vi "Requirement Coverage.vi"() -> ()   [LabVIEW 2013]
uses:
  <vilib>/addons/_JKI Toolkits/Caraya/classes/Test/Test.lvclass
  <vilib>/LabVIEW Open Source Project/MQTT TCP Connection/MQTT_TCP/Connection/TCPConnection.lvclass
  source/Server class/Server.lvclass
  <vilib>/LabVIEW Open Source Project/MQTT Connection/MQTT_Base/Base Class/MQTT_Base.lvclass
panel:
  out "error out":errorcluster
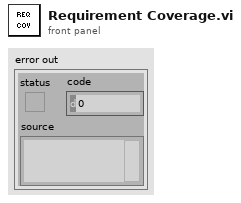
[diagram p1: front panel]
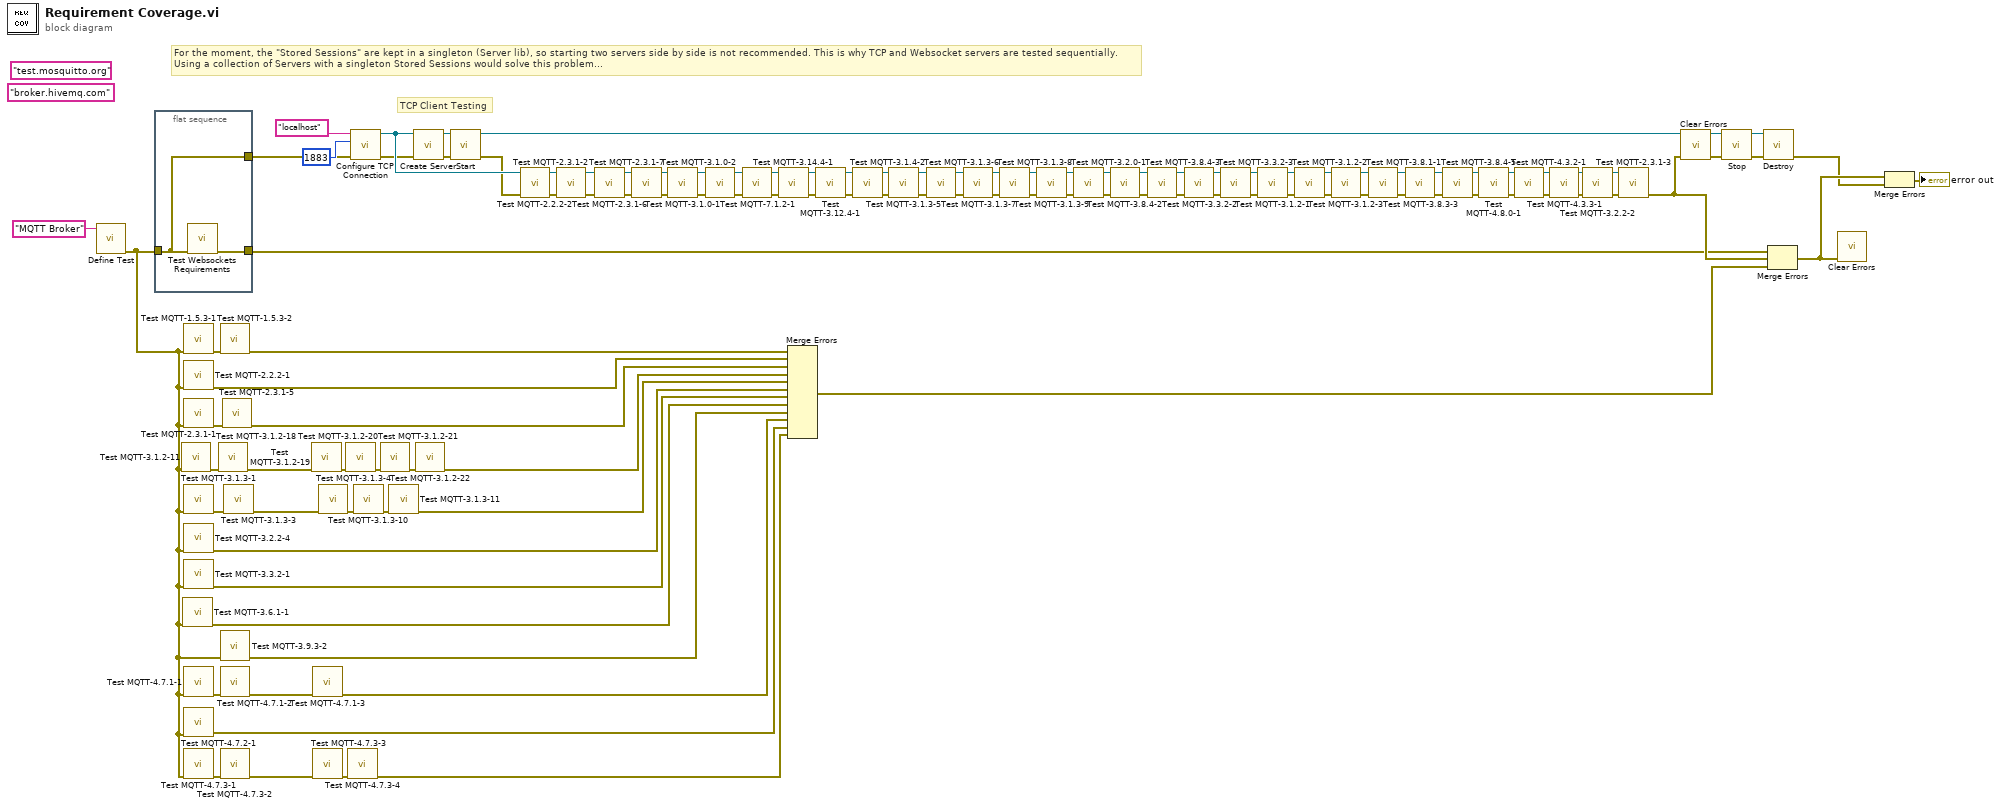
[diagram p0: block diagram]
diagram:
  (unwired) "test.mosquitto.org" ("address (localhost)")
  (unwired) "broker.hivemq.com" ("address (localhost)")
  # "For the moment, the \"Stored Sessions\" are kept in a singleton (Server lib), so starting two servers side by side is not recommended. This is why TCP and Websocket servers are tested sequentially.\nUsing a collection of Servers with a singleton Stored Sessions would solve this problem..."
  # "TCP Client Testing"
  n1 = call <vilib>:"Define Test.vi"("Label (VI Title)"="MQTT Broker" ("address (localhost)")) -> ("error out"=w4:errorcluster)  [unwired: 9 in, 1 out]
  n2 = flat-sequence {
    tunnel: w4 -> [w109]
    tunnel: [w110] -> w3
    tunnel: [w109] -> w2
    frame #0 {
      n3 = call "Test Websockets Requirements.vi"("error in (no error)"=w109) -> ("error out"=w110:errorcluster)  [unwired: 10 in]
    }
  }
  n4 = call "Test MQTT-3.1.2-11.vi"("error in (no error)"=w4) -> ("error out"=w94:errorcluster)  [unwired: 10 in]
  n5 = call "Test MQTT-3.6.1-1.vi"("error in (no error)"=w4) -> ("error out"=w98:errorcluster)  [unwired: 10 in]
  n6 = call "Test MQTT-1.5.3-1.vi"("error in (no error)"=w4) -> ("error out"=w107:errorcluster)  [unwired: 10 in]
  n7 = call "Test MQTT-2.2.2-1.vi"("error in (no error)"=w4) -> ("error out"=w82:errorcluster)  [unwired: 10 in]
  n8 = call "Test MQTT-2.3.1-1.vi"("error in (no error)"=w4) -> ("error out"=w83:errorcluster)  [unwired: 10 in]
  n9 = call "Test MQTT-3.1.3-1.vi"("error in (no error)"=w4) -> ("error out"=w87:errorcluster)  [unwired: 10 in]
  n10 = call "Test MQTT-3.2.2-4.vi"("error in (no error)"=w4) -> ("error out"=w97:errorcluster)  [unwired: 10 in]
  n11 = call "Test MQTT-3.3.2-1.vi"("error in (no error)"=w4) -> ("error out"=w81:errorcluster)  [unwired: 10 in]
  n12 = call "Test MQTT-4.7.1-1.vi"("error in (no error)"=w4) -> ("error out"=w102:errorcluster)  [unwired: 10 in]
  n13 = call "Test MQTT-4.7.2-1.vi"("error in (no error)"=w4) -> ("error out"=w96:errorcluster)  [unwired: 10 in]
  n14 = call "Test MQTT-4.7.3-1.vi"("error in (no error)"=w4) -> ("error out"=w105:errorcluster)  [unwired: 10 in]
  n15 = call "Test MQTT-3.1.2-18.vi"("error in (no error)"=w94) -> ("error out"=w93:errorcluster)  [unwired: 10 in]
  n16 = call "Test MQTT-1.5.3-2.vi"("error in (no error)"=w107) -> ("error out"=w108:errorcluster)  [unwired: 10 in]
  n17 = call "Test MQTT-3.9.3-2.vi"("error in (no error)"=w4) -> ("error out"=w106:errorcluster)  [unwired: 10 in]
  n18 = call "Test MQTT-4.7.1-2.vi"("error in (no error)"=w102) -> ("error out"=w101:errorcluster)  [unwired: 10 in]
  n19 = call "Test MQTT-4.7.3-2.vi"("error in (no error)"=w105) -> ("error out"=w104:errorcluster)  [unwired: 10 in]
  n20 = call "Test MQTT-2.3.1-5.vi"("error in (no error)"=w83) -> ("error out"=w84:errorcluster)  [unwired: 10 in]
  n21 = call "Test MQTT-3.1.3-3.vi"("error in (no error)"=w87) -> ("error out"=w86:errorcluster)  [unwired: 10 in]
  n22 = call "Test MQTT-3.1.2-19.vi"("error in (no error)"=w93) -> ("error out"=w91:errorcluster)  [unwired: 10 in]
  n23 = call "Test MQTT-4.7.1-3.vi"("error in (no error)"=w101) -> ("error out"=w100:errorcluster)  [unwired: 10 in]
  n24 = call "Test MQTT-4.7.3-3.vi"("error in (no error)"=w104) -> ("error out"=w103:errorcluster)  [unwired: 10 in]
  n25 = call "Test MQTT-3.1.3-4.vi"("error in (no error)"=w86) -> ("error out"=w80:errorcluster)  [unwired: 10 in]
  n26 = call "Test MQTT-3.1.2-20.vi"("error in (no error)"=w91) -> ("error out"=w92:errorcluster)  [unwired: 10 in]
  n27 = call "Test MQTT-4.7.3-4.vi"("error in (no error)"=w103) -> ("error out"=w95:errorcluster)  [unwired: 10 in]
  n28 = call <vilib>:"Configure TCP Connection.vi"("error in (no error)"=w2, "remote port (80)"=u16 1883, "address (localhost)"="localhost") -> ("error out"=w1:errorcluster, "TCPConnection"=w77:refnum<class "TCPConnection.lvclass">)  [unwired: 7 in]
  n29 = call "Test MQTT-3.1.3-10.vi"("error in (no error)"=w80) -> ("error out"=w85:errorcluster)  [unwired: 10 in]
  n30 = call "Test MQTT-3.1.2-21.vi"("error in (no error)"=w92) -> ("error out"=w90:errorcluster)  [unwired: 10 in]
  n31 = call "Test MQTT-3.1.3-11.vi"("error in (no error)"=w85) -> ("error out"=w88:errorcluster)  [unwired: 10 in]
  n32 = call "Create Server.vi"("error in (no error)"=w1, "Connection Configuration"=w77) -> ("error out"=w76:errorcluster, "Server"=w75:refnum<class "Server.lvclass">)  [unwired: 8 in]
  n33 = call "Test MQTT-3.1.2-22.vi"("error in (no error)"=w90) -> ("error out"=w89:errorcluster)  [unwired: 10 in]
  n34 = call <vilib>:"Start.vi"("error in (no error)"=w76, "MQTT_Base in"=w75) -> ("error out"=w16:errorcluster, "MQTT_Base out"=w7:refnum<class "Server.lvclass">)  [unwired: 7 in, 1 out]
  n35 = call "Test MQTT-2.2.2-2.vi"("error in (no error)"=w16, "Connection Config"=w77) -> ("error out"=w68:errorcluster, "Connection Config dup"=w65:refnum<class "TCPConnection.lvclass">)  [unwired: 8 in]
  n36 = call "Test MQTT-2.3.1-2.vi"("error in (no error)"=w68, "Connection Config"=w65) -> ("error out"=w71:errorcluster, "Connection Config dup"=w17:refnum<class "TCPConnection.lvclass">)  [unwired: 8 in]
  n37 = call "Test MQTT-2.3.1-6.vi"("error in (no error)"=w71, "Connection Config"=w17) -> ("error out"=w70:errorcluster, "Connection Config dup"=w64:refnum<class "TCPConnection.lvclass">)  [unwired: 8 in]
  n38 = call "Test MQTT-2.3.1-7.vi"("error in (no error)"=w70, "Connection Config"=w64) -> ("error out"=w67:errorcluster, "Connection Config dup"=w63:refnum<class "TCPConnection.lvclass">)  [unwired: 8 in]
  n39 = call "Test MQTT-3.1.0-1.vi"("error in (no error)"=w67, "Connection Config"=w63) -> ("error out"=w69:errorcluster, "Connection Config dup"=w62:refnum<class "TCPConnection.lvclass">)  [unwired: 8 in]
  n40 = call "Test MQTT-3.1.0-2.vi"("error in (no error)"=w69, "Connection Config"=w62) -> ("error out"=w66:errorcluster, "Connection Config dup"=w61:refnum<class "TCPConnection.lvclass">)  [unwired: 8 in]
  n41 = call "Test MQTT-7.1.2-1.vi"("error in (no error)"=w66, "Connection Config"=w61) -> ("error out"=w60:errorcluster, "Connection Config dup"=w58:refnum<class "TCPConnection.lvclass">)  [unwired: 8 in]
  n42 = call "Test MQTT-3.14.4-1.vi"("error in (no error)"=w60, "Connection Config"=w58) -> ("error out"=w59:errorcluster, "Connection Config dup"=w51:refnum<class "TCPConnection.lvclass">)  [unwired: 8 in]
  n43 = Merge Errors(w108, w82, w84, w89, w88, w97, w81, w98, w106, w100, w96, w95) -> (w79:errorcluster)
  n44 = call "Test MQTT-3.12.4-1.vi"("error in (no error)"=w59, "Connection Config"=w51) -> ("error out"=w53:errorcluster, "Connection Config dup"=w50:refnum<class "TCPConnection.lvclass">)  [unwired: 8 in]
  n45 = call "Test MQTT-3.1.4-2.vi"("error in (no error)"=w53, "Connection Config"=w50) -> ("error out"=w52:errorcluster, "Connection Config dup"=w49:refnum<class "TCPConnection.lvclass">)  [unwired: 8 in]
  n46 = call "Test MQTT-3.1.3-5.vi"("error in (no error)"=w52, "Connection Config"=w49) -> ("error out"=w56:errorcluster, "Connection Config dup"=w48:refnum<class "TCPConnection.lvclass">)  [unwired: 8 in]
  n47 = call "Test MQTT-3.1.3-6.vi"("error in (no error)"=w56, "Connection Config"=w48) -> ("error out"=w55:errorcluster, "Connection Config dup"=w47:refnum<class "TCPConnection.lvclass">)  [unwired: 8 in]
  n48 = call "Test MQTT-3.1.3-7.vi"("error in (no error)"=w55, "Connection Config"=w47) -> ("error out"=w54:errorcluster, "Connection Config dup"=w46:refnum<class "TCPConnection.lvclass">)  [unwired: 8 in]
  n49 = call "Test MQTT-3.1.3-8.vi"("error in (no error)"=w54, "Connection Config"=w46) -> ("error out"=w57:errorcluster, "Connection Config dup"=w44:refnum<class "TCPConnection.lvclass">)  [unwired: 8 in]
  n50 = call "Test MQTT-3.1.3-9.vi"("error in (no error)"=w57, "Connection Config"=w44) -> ("error out"=w45:errorcluster, "Connection Config dup"=w43:refnum<class "TCPConnection.lvclass">)  [unwired: 8 in]
  n51 = call "Test MQTT-3.2.0-1.vi"("error in (no error)"=w45, "Connection Config"=w43) -> ("error out"=w39:errorcluster, "Connection Config dup"=w40:refnum<class "TCPConnection.lvclass">)  [unwired: 8 in]
  n52 = call "Test MQTT-3.8.4-2.vi"("error in (no error)"=w39, "Connection Config"=w40) -> ("error out"=w41:errorcluster, "Connection Config dup"=w42:refnum<class "TCPConnection.lvclass">)  [unwired: 8 in]
  n53 = call "Test MQTT-3.8.4-3.vi"("error in (no error)"=w41, "Connection Config"=w42) -> ("error out"=w37:errorcluster, "Connection Config dup"=w38:refnum<class "TCPConnection.lvclass">)  [unwired: 8 in]
  n54 = call "Test MQTT-3.3.2-2.vi"("error in (no error)"=w37, "Connection Config"=w38) -> ("error out"=w36:errorcluster, "Connection Config dup"=w35:refnum<class "TCPConnection.lvclass">)  [unwired: 8 in]
  n55 = call "Test MQTT-3.3.2-3.vi"("error in (no error)"=w36, "Connection Config"=w35) -> ("error out"=w34:errorcluster, "Connection Config dup"=w33:refnum<class "TCPConnection.lvclass">)  [unwired: 8 in]
  n56 = call "Test MQTT-3.1.2-1.vi"("error in (no error)"=w34, "Connection Config"=w33) -> ("error out"=w32:errorcluster, "Connection Config dup"=w31:refnum<class "TCPConnection.lvclass">)  [unwired: 8 in]
  n57 = call "Test MQTT-3.1.2-2.vi"("error in (no error)"=w32, "Connection Config"=w31) -> ("error out"=w27:errorcluster, "Connection Config dup"=w26:refnum<class "TCPConnection.lvclass">)  [unwired: 8 in]
  n58 = call "Test MQTT-3.1.2-3.vi"("error in (no error)"=w27, "Connection Config"=w26) -> ("error out"=w29:errorcluster, "Connection Config dup"=w25:refnum<class "TCPConnection.lvclass">)  [unwired: 8 in]
  n59 = call "Test MQTT-3.8.1-1.vi"("error in (no error)"=w29, "Connection Config"=w25) -> ("error out"=w28:errorcluster, "Connection Config dup"=w24:refnum<class "TCPConnection.lvclass">)  [unwired: 8 in]
  n60 = call "Test MQTT-3.8.3-3.vi"("error in (no error)"=w28, "Connection Config"=w24) -> ("error out"=w30:errorcluster, "Connection Config dup"=w23:refnum<class "TCPConnection.lvclass">)  [unwired: 8 in]
  n61 = call "Test MQTT-3.8.4-5.vi"("error in (no error)"=w30, "Connection Config"=w23) -> ("error out"=w18:errorcluster, "Connection Config dup"=w19:refnum<class "TCPConnection.lvclass">)  [unwired: 8 in]
  n62 = call "Test MQTT-4.8.0-1.vi"("error in (no error)"=w18, "Connection Config"=w19) -> ("error out"=w12:errorcluster, "Connection Config dup"=w13:refnum<class "TCPConnection.lvclass">)  [unwired: 8 in]
  n63 = call "Test MQTT-4.3.2-1.vi"("error in (no error)"=w12, "Connection Config"=w13) -> ("error out"=w9:errorcluster, "Connection Config dup"=w11:refnum<class "TCPConnection.lvclass">)  [unwired: 8 in]
  n64 = call "Test MQTT-4.3.3-1.vi"("error in (no error)"=w9, "Connection Config"=w11) -> ("error out"=w8:errorcluster, "Connection Config dup"=w10:refnum<class "TCPConnection.lvclass">)  [unwired: 8 in]
  n65 = call "Test MQTT-3.2.2-2.vi"("error in (no error)"=w8, "Connection Config"=w10) -> ("error out"=w14:errorcluster, "Connection Config dup"=w15:refnum<class "TCPConnection.lvclass">)  [unwired: 8 in]
  n66 = call "Test MQTT-2.3.1-3.vi"("error in (no error)"=w14, "Connection Configuration"=w15) -> ("error out"=w6:errorcluster)  [unwired: 8 in, 1 out]
  n67 = call <vilib>:"Clear Errors.vi"("error in (no error)"=w6) -> ("error out"=w5:errorcluster)  [unwired: 6 in]
  n68 = call <vilib>:"Stop.vi"("error in (no error)"=w5, "MQTT_Base in"=w7) -> ("error out"=w74:errorcluster, "MQTT_Base out"=w73:refnum<class "Server.lvclass">)  [unwired: 7 in, 1 out]
  n69 = call <vilib>:"Destroy.vi"("error in (no error)"=w74, "MQTT_Base in"=w73) -> ("error out"=w72:errorcluster)  [unwired: 8 in, 1 out]
  n70 = Merge Errors(w3, w6, w79) -> (w78:errorcluster)
  n71 = call <vilib>:"Clear Errors.vi"("error in (no error)"=w78) -> ()  [unwired: 6 in, 1 out]
  n72 = Merge Errors(w78, w72) -> (→"error out":errorcluster)
